vi "Connect CO3000.vi"(8 "error in (no error)":errorcluster caption="에러 입력(에러 없음)", 10 "VISA resource name":refnum<visa-resource-name>, 11 "Instrument Manager 입력":refnum<class "Instrument Manager.lvclass">) -> (0 "error out":errorcluster caption="에러 출력", 3 "Instrument Manager 출력":refnum<class "Instrument Manager.lvclass">)   [LabVIEW 2023, in "Instrument Manager.lvclass"]
uses:
  Instrument Manager.lvclass
  Instrument Manager.lvclass/Instrument Manager.ctl
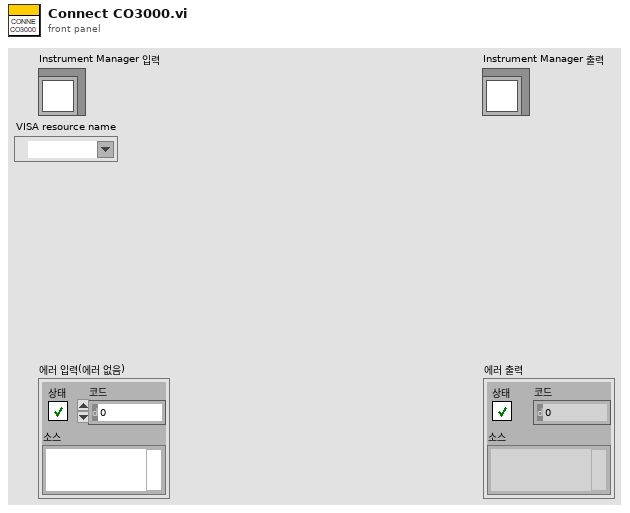
[diagram p1: front panel]
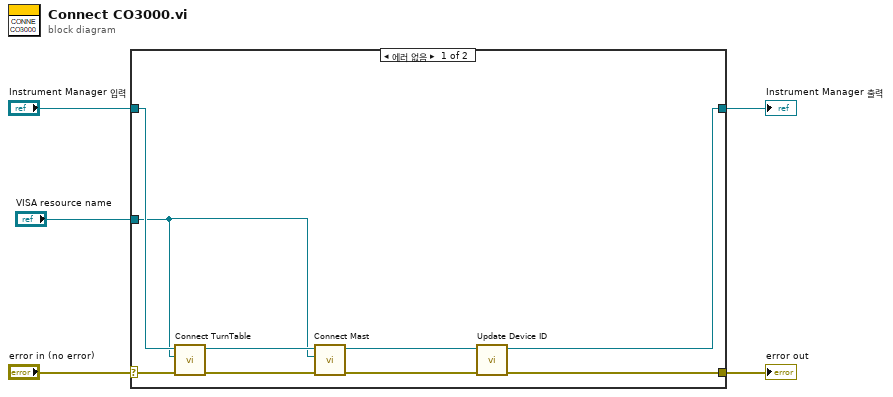
[diagram p0: block diagram]
diagram:
  n1 = case shown="에러 없음" "error in (no error)" {
    selector: "error in (no error)" -> [w14 w16]
    tunnel: [w6 w16] -> w4
    tunnel: [w7 w15] -> w2
    tunnel: "Instrument Manager 입력" -> [w12 w15]
    tunnel: "VISA resource name" -> [w10 _]
    frame No Error {
      n2 = call "Connect TurnTable.vi"("error in (no error)"=w14, "VISA resource name"=w10, "Instrument Manager 입력"=w12) -> ("error out"=w13:errorcluster, "Instrument Manager 출력"=w11:refnum<class "Instrument Manager.lvclass">)  [unwired: 7 in]
      n3 = call "Connect Mast.vi"("error in (no error)"=w13, "VISA resource name"=w10, "Instrument Manager 입력"=w11) -> ("error out"=w9:errorcluster, "Instrument Manager 출력"=w8:refnum<class "Instrument Manager.lvclass">)  [unwired: 7 in]
      n4 = call "Update Device ID.vi"("error in (no error)"=w9, "Instrument Manager 입력"=w8) -> ("error out"=w6:errorcluster, "Instrument Manager 출력"=w7:refnum<class "Instrument Manager.lvclass">)  [unwired: 8 in]
    }
    frame Error {
    }
  }
  "error out" <- w4
  "Instrument Manager 출력" <- w2
